vi "test_Basic Write.vi"(8 "error in (no error)":errorcluster, 11 "Scalar Channels Testing in":refnum<class "FPGA Addon Scalar Channels System Tests.lvclass">) -> (0 "error out":errorcluster, 3 "Scalar Channels Testing out":refnum<class "FPGA Addon Scalar Channels System Tests.lvclass">)   [LabVIEW 2020, in "FPGA Addon Scalar Channels System Tests.lvclass"]
uses:
  FPGA Addon Scalar Channels System Tests.lvclass
  C:/Users/nitest/Desktop/Git 2020/niveristand-fpga-addon-custom-device/Source/Tests/FPGA Addon Test Class/FPGA Addon Test Class.lvclass
  C:/Program Files (x86)/National Instruments/LabVIEW 2020/vi.lib/NI/VeriStand Custom Device Testing Tools/VeriStandTestCase/VeriStandTestCase.lvclass
  FPGA Addon Test Class/FPGA Addon Test Class.lvclass/FPGA Addon Test Class.ctl
  <vilib>/NI VeriStand/Execution/Workspace/NI VeriStand - Set Single Channel Value.vi
  <vilib>/NI VeriStand/Execution/Workspace/NI_VS Workspace ExecutionAPI.lvlib
  FPGA Addon Test Class/FPGA Addon Test Class.lvclass
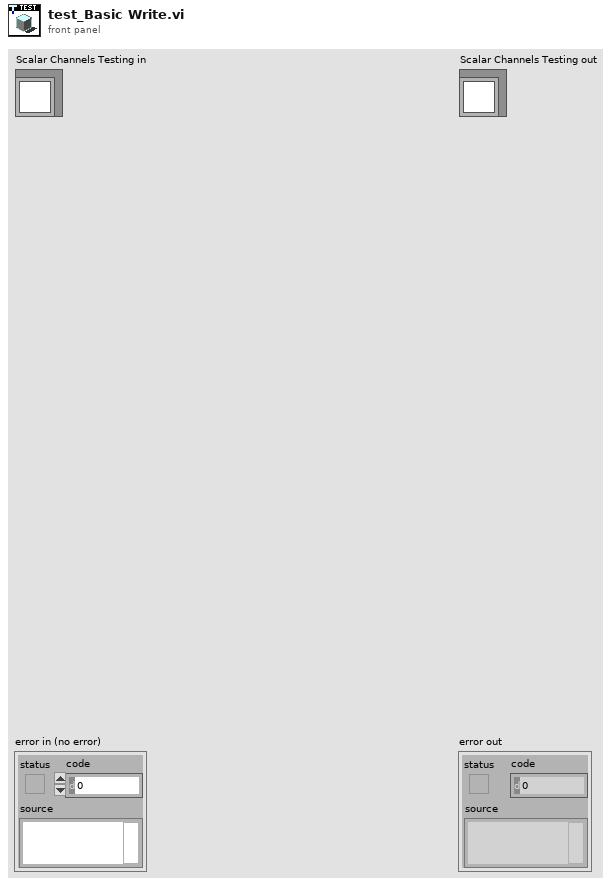
[diagram p1: front panel]
types:
  T1 = typedef "NI_VS Workspace ExecutionAPI.lvlib/WorkspaceAPI.ctl" = refnum<k24>
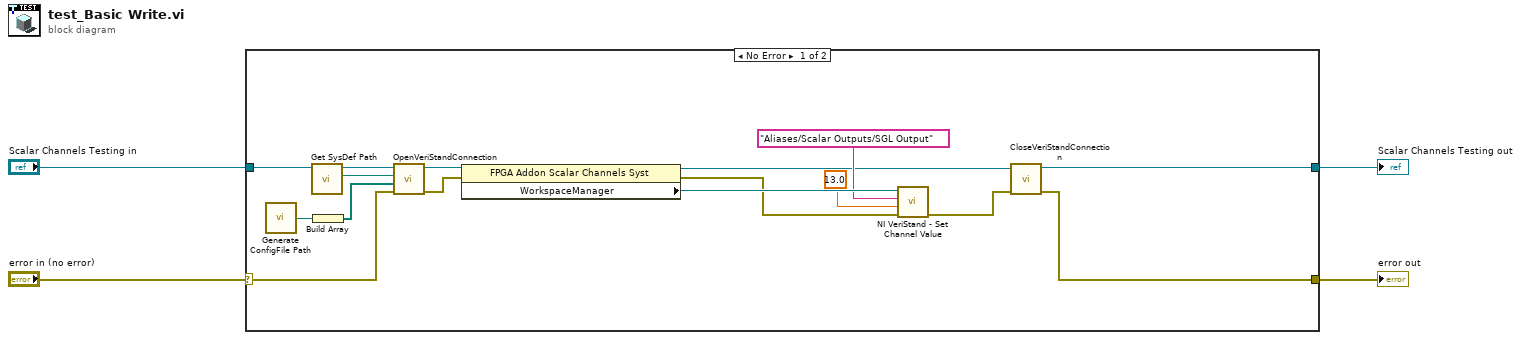
[diagram p0: block diagram]
diagram:
  n1 = case shown="No Error" "error in (no error)" {
    selector: "error in (no error)" -> [w10 w22]
    tunnel: [w19 w22] -> w3
    tunnel: [w20 w21] -> w1
    tunnel: "Scalar Channels Testing in" -> [w9 w21]
    frame No Error {
      n2 = call "Generate ConfigFile Path.vi"() -> ("ConfigFile path"=w6:path)
      n3 = call "Get SysDef Path.vi"("Scalar Channels Testing in"=w9) -> ("SysDef Path"=w7:path, "Scalar Channels Testing out"=w8:refnum<class "FPGA Addon Scalar Channels System Tests.lvclass">)  [unwired: 9 in]
      n4 = Build Array(w6) -> (w5:path[])
      n5 = call-dynamic "OpenVeriStandConnection.vi"("error in (no error)"=w10, "overrides files"=w5, "System Definition File"=w7, "VeriStand Test Case in"=w8) -> ("error out"=w17:errorcluster, "VeriStand Test Case out"=w18:refnum<class "FPGA Addon Scalar Channels System Tests.lvclass">)  [unwired: 5 in, 1 out]
      n6 = property class="FPGA Addon Scalar Channels Syst"(reference=w18, error in=w17) -> (reference out=w12:refnum<class "FPGA Addon Scalar Channels System Tests.lvclass">, error out=w13:errorcluster, "WorkspaceManager"=w16:T1)
      n7 = call-poly <vilib>:"NI VeriStand - Set Channel Value.vi"("error in (no error)"=w13, "Value"=13.0, "Channel"="Aliases/Scalar Outputs/SGL Output", "WorkspaceManager in"=w16) -> ("error out"=w11:errorcluster)  [unwired: 6 in, 1 out]
      n8 = call-dynamic "CloseVeriStandConnection.vi"("error in (no error)"=w11, "VeriStand Test Case in"=w12) -> ("error out"=w19:errorcluster, "VeriStand Test Case out"=w20:refnum<class "FPGA Addon Scalar Channels System Tests.lvclass">)  [unwired: 8 in]
    }
    frame Error {
    }
  }
  "error out" <- w3
  "Scalar Channels Testing out" <- w1
